vi "Update CLFN in LV2014 Deploy.vi"() -> ()   [LabVIEW 2014]
uses:
  <vilib>/Utility/lvfile.llb/FT_FileTypes.ctl
  <vilib>/Utility/traverseref.llb/TRef TravTarget.ctl
  <vilib>/Utility/error.llb/Error Cluster From Error Code.vi
  <vilib>/ErrorRing/Error Ring.xnode
  <vilib>/Utility/traverseref.llb/VI Scripting - Traverse.lvlib
  <vilib>/Utility/lvfile.llb/NI_FileType.lvlib
panel:
  out "Total Files":i32
  out "File #":i32
  out "Pass #":i32
  out "Project file":path
  out "Updated VIs":path[](array[path])
  out "error out":errorcluster
  # "Progress"
  # "IMPORTANT NOTICE:\nTHIS VI MUST BE SAVED AND RUN IN LABVIEW 2014."
  # "Run this VI to set proper path to the CalcExpress Engine DLL\nin the Call Library Function Nodes (CLFN) within the\nCalcExpress Deployment for LabVIEW 2014 project."
  # "CalcExpress Toolkit\nCopyright (c) 2000-2026 Konstantin Shifershteyn"
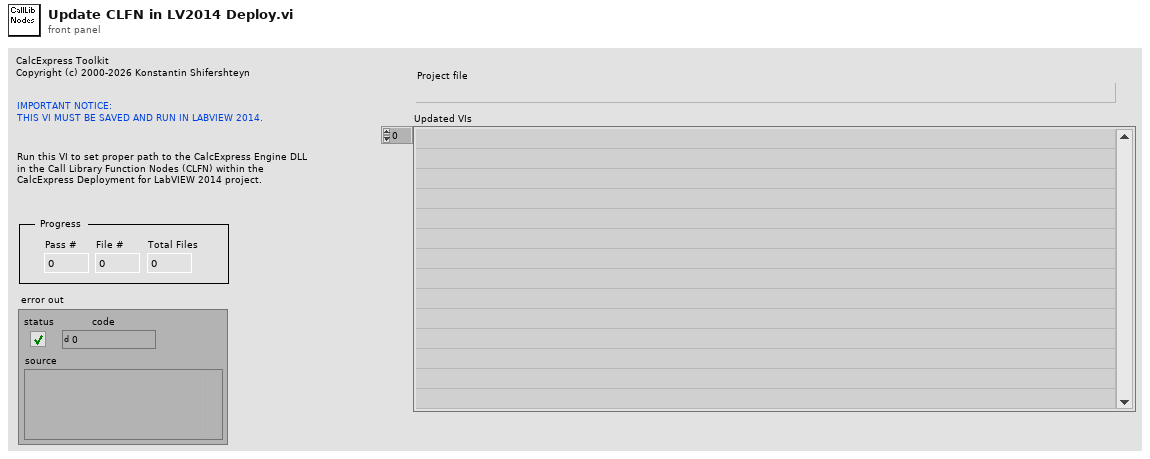
[diagram p1: front panel]
types:
  T1 = typedef "NI_FileType.lvlib/FT_FileTypes.ctl" = enum32{"Invalid file/path", "Unknown type", "Instrument", "Control", "Polymorphic VI", "Project", "Library", "LVClass", "XControl", "XNode", "CIN", "Run-time menu", "Palette menu", "LLB", "Shortcut", "Directory", "Class Private Data Control", "Statechart", "MathScript .m file", "Ladder Diagram", "LVLibp"}
  T2 = typedef "TRef TravTarget.ctl" = enum16{"FP", "BD", "Other"}
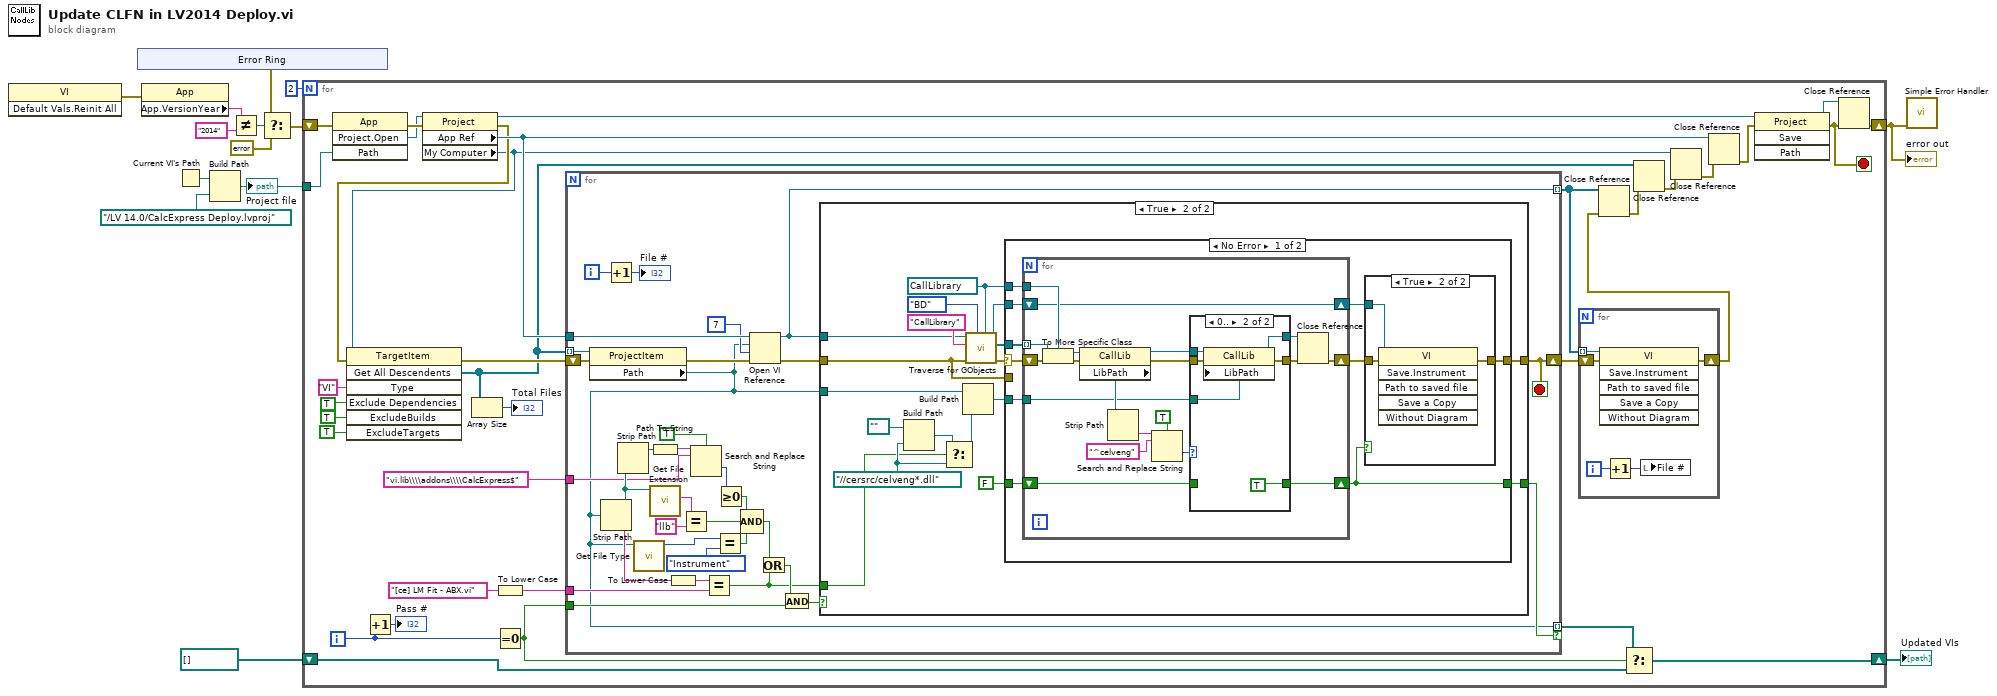
[diagram p0: block diagram]
diagram:
  n1 = invoke class="VI" method="Default Vals.Reinit All"() -> (error out=w1:errorcluster)  [unwired: 3 in, 2 out]
  n2 = xnode "Error Ring"() -> ("error out"=w8:errorcluster)
  n3 = property class="App"(error in=w1) -> ("App.VersionYear"=w11:string)  [unwired: 1 in, 2 out]
  n4 = Current VI's Path() -> (path=w4:path)
  n5 = Build Path(base path=w4, name or relative path=path "../LV 14.0/CalcExpress Deploy.lvproj") -> (appended path=w2:path)
  "Project file" <- w2
  n6 = Not Equal?(x=w11, y="2014") -> (x != y?=w9:bool)
  n7 = Select(t=w8, s=w9, f=errorcluster {"status"=FALSE, "code"=0, "source"=""}) -> (s? t:f=w7:errorcluster)
  n8 = for {
    N: 2 -> [_]
    shift-right: [w34] -> w5
    shift-left: w7 -> [w31]
    shift-right: [w28] -> w13
    shift-left: path[] [] -> [w27]
    tunnel: w2 -> [w24]
    i -> [w17]
    stop <- w30 stop-if-true
    n9 = invoke class="App" method="Project.Open"(error in=w31, "Path"=w24) -> (error out=w41:errorcluster, "Project:Open"=w32:refnum<vi>)  [unwired: 2 in, 2 out]
    n10 = Increment(x=w17) -> (x+1=→"Pass #":i32)
    n11 = property class="Project"(reference=w32, error in=w41) -> (error out=w23:errorcluster, "App Ref"=w38:refnum<vi>, "My Computer"=w22:refnum<vi>)  [unwired: 1 out]
    n12 = invoke class="TargetItem" method="Get All Descendents"(reference=w22, error in=w23, "Type"="VI", "Exclude Dependencies"=TRUE, "ExcludeBuilds"=TRUE, "ExcludeTargets"=TRUE) -> (error out=w46:errorcluster, "All Descendents"=w16:refnum<vi>[])  [unwired: 1 in, 5 out]
    n13 = Array Size(array=w16) -> (size(s)=→"Total Files":i32)
    n14 = To Lower Case(string="[ce] LM Fit - ABX.vi") -> (all lower case string=w20:string)
    n15 = Equal To 0?(x=w17) -> (x = 0?=w26:bool)
    n16 = for {
      tunnel: w16 -> [w85] mode=indexing
      shift-right: [w82] -> w37
      shift-left: w46 -> [w84]
      tunnel: [w56] -> w29 mode=indexing if=w83
      tunnel: w38 -> [w81]
      tunnel: [w77] -> w33 mode=indexing
      tunnel: w26 -> [w75]
      tunnel: w20 -> [w59]
      tunnel: "vi.lib\\\\addons\\\\CalcExpress$" -> [w57]
      i -> [w54]
      stop <- w82 stop-if-true
      n17 = property class="ProjectItem"(reference=w85, error in=w84) -> (error out=w79:errorcluster, "Path"=w56:path)  [unwired: 1 out]
      n18 = Strip Path(path=w56) -> (stripped path=w70:path, name=w61:string)
      n19 = Increment(x=w54) -> (x+1=→"File #":i32)
      n20 = Strip Path(path=w70) -> (stripped path=w69:path)  [unwired: 1 out]
      n21 = call <vilib>:"Get File Type.vi"("path"=w56) -> ("file type"=w64:T1)  [unwired: 8 in, 2 out]
      n22 = Path To String(path=w69) -> (string=w68:string)
      n23 = call <vilib>:"Get File Extension.vi"("file"=w70) -> ("lowercase file extension"=w66:string)  [unwired: 7 in, 3 out]
      n24 = To Lower Case(string=w61) -> (all lower case string=w62:string)
      n25 = Equal?(x=w66, y="llb") -> (x = y?=w71:bool)
      n26 = Search and Replace String(case sensitive?=TRUE, input string=w68, search string=w57) -> (offset past replacement=w74:i32)  [unwired: 5 in, 3 out]
      n27 = Equal?(x=w62, y=w59) -> (x = y?=w55:bool)
      n28 = Equal?(x=w64, y=FT_FileTypes."Instrument" ("file type")) -> (x = y?=w63:bool)
      n29 = Greater Or Equal To 0?(x=w74) -> (x >= 0?=w73:bool)
      n30 = Compound Arithmetic op=AND(w73, w71, w63) -> (w60:bool)
      n31 = Open VI Reference(application reference (local)=w81, vi path=w56, options=7, error in (no error)=w79) -> (vi reference=w77:refnum<vi>, error out=w78:errorcluster)  [unwired: 2 in]
      n32 = Or(x=w60, y=w55) -> (x .or. y?=w58:bool)
      n33 = And(x=w58, y=w75) -> (x .and. y?=w76:bool)
      n34 = case shown="True" w76 {
        tunnel: [w86 w97] -> w82
        tunnel: w78 -> [w86 w92]
        tunnel: [_ w99] -> w83
        tunnel: w77 -> [_ w93]
        tunnel: w56 -> [_ w94]
        tunnel: w55 -> [_ w87]
        frame False {
        }
        frame True {
          w90 = path "../../cersrc/celveng*.dll" ("default relative path to DLL")
          w104 = refnum<vi> refnum ("Other Refnum")
          n35 = Build Path(base path=path "..", name or relative path=w90) -> (appended path=w91:path)
          n36 = Select(t=w91, s=w87, f=w90) -> (s? t:f=w88:path)
          n37 = Build Path(base path=w94, name or relative path=w88) -> (appended path=w96:path)
          n38 = call <vilib>:"Traverse for GObjects.vi"("Other Refnum"=w104, "Traverse Target"=TRef_TravTarget."BD", "error in (no error)"=w92, "Class Name"="CallLibrary", "VI Refnum"=w93) -> ("error out"=w98:errorcluster, "References"=w102:refnum<vi>[], "dup VI Refnum"=w103:refnum<vi>)  [unwired: 3 in, 1 out]
          n39 = case shown="No Error" w98 {
            selector: w98 -> [w111 _]
            tunnel: w96 -> [w114 _]
            tunnel: w104 -> [w113 _]
            tunnel: w103 -> [w112 _]
            tunnel: w102 -> [w107 _]
            tunnel: [w106 w147] -> w97
            tunnel: [w108 _] -> w99
            tunnel: w92 -> [_ w147]
            tunnel: FALSE -> [w105 _]
            frame No Error {
              n40 = for {
                shift-right: [w124] -> w109
                shift-left: w111 -> [w137]
                tunnel: w107 -> [w136] mode=indexing
                tunnel: w113 -> [w135]
                shift-right: [w129] -> w110
                shift-left: w112 -> [w129]
                shift-right: [w128] -> w108
                shift-left: w105 -> [w127]
                tunnel: w114 -> [w126]
                n41 = To More Specific Class(target class=w135, reference=w136, error in=w137) -> (specific class reference=w133:refnum<vi>, error out=w134:errorcluster)
                n42 = property class="CallLib"(reference=w133, error in=w134) -> (reference out=w130:refnum<vi>, error out=w131:errorcluster, "LibPath"=w132:path)
                n43 = Strip Path(path=w132) -> (name=w122:string)  [unwired: 1 out]
                n44 = Search and Replace String(case sensitive?=TRUE, input string=w122, search string="^celveng") -> (offset past replacement=w121:i32)  [unwired: 5 in, 3 out]
                n45 = case shown="0.." w121 {
                  tunnel: [w140 w144] -> w125
                  tunnel: w131 -> [w140 w146]
                  tunnel: w130 -> [w139 w145]
                  tunnel: [w139 w143] -> w123
                  tunnel: [w138 TRUE] -> w128
                  tunnel: w127 -> [w138 _]
                  tunnel: w126 -> [_ w141]
                  frame ..-1 {
                  }
                  frame 0.. {
                    n46 = property class="CallLib"(reference=w145, error in=w146, "LibPath"=w141) -> (reference out=w143:refnum<vi>, error out=w144:errorcluster)
                  }
                }
                n47 = Close Reference(reference=w123, error in (no error)=w125) -> (error out=w124:errorcluster)
              }
              n48 = case shown="True" w108 {
                tunnel: w110 -> [_ w118]
                tunnel: w109 -> [w115 w117]
                tunnel: [w115 w116] -> w106
                frame False {
                }
                frame True {
                  n49 = invoke class="VI" method="Save.Instrument"(reference=w118, error in=w117) -> (error out=w116:errorcluster)  [unwired: 4 in, 5 out]
                }
              }
            }
            frame Error {
            }
          }
        }
      }
    }
    n50 = for {
      tunnel: w33 -> [w52] mode=indexing
      shift-right: [w50] -> w25
      shift-left: w37 -> [w51]
      i -> [w49]
      n51 = invoke class="VI" method="Save.Instrument"(reference=w52, error in=w51) -> (error out=w50:errorcluster)  [unwired: 4 in, 5 out]
      n52 = Increment(x=w49) -> (x+1=w48:i32)
      n53 = local write "File #"(w48) -> ()
    }
    n54 = Close Reference(reference=w33, error in (no error)=w25) -> (error out=w40:errorcluster)
    n55 = Select(t=w29, s=w26, f=w27) -> (s? t:f=w28:path[])
    n56 = Close Reference(reference=w16, error in (no error)=w40) -> (error out=w42:errorcluster)
    n57 = Close Reference(reference=w22, error in (no error)=w42) -> (error out=w39:errorcluster)
    n58 = Close Reference(reference=w38, error in (no error)=w39) -> (error out=w35:errorcluster)
    n59 = invoke class="Project" method="Save"(reference=w32, error in=w35) -> (reference out=w36:refnum<vi>, error out=w30:errorcluster)  [unwired: 2 in, 2 out]
    n60 = Close Reference(reference=w36, error in (no error)=w30) -> (error out=w34:errorcluster)
  }
  "error out" <- w5
  "Updated VIs" <- w13
  n61 = call <vilib>:"Simple Error Handler.vi"("error in (no error)"=w5) -> ()  [unwired: 4 in, 5 out]
